vi "Update Overlay.vi"(8 "error in":errorcluster, 11 "BigMAQ in":refnum<class "BigMAQ.lvclass">) -> (0 "error out":errorcluster, 2 "Overlays":T1[](array[typedef]), 3 "BigMAQ out":refnum<class "BigMAQ.lvclass">)   [LabVIEW 2019, in "BigMAQ.lvclass"]
uses:
  BigMAQ.lvclass
  Overlay.ctl
  BigMAQ.lvclass/BigMAQ.ctl
  <vilib>/LabVIEW Open Source Project/Unicity/RandomStringGenerator/RandomStringGenerator.lvclass
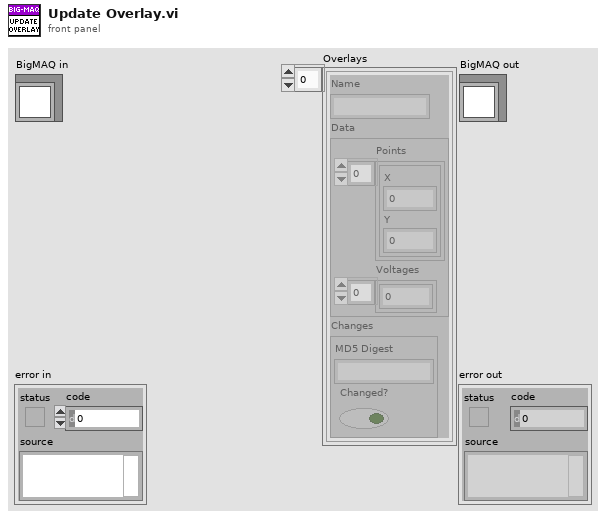
[diagram p1: front panel]
types:
  T1 = typedef "BigMAQ.lvclass/Overlay.ctl" = cluster{"Name":string, "Data":cluster{"Points":cluster{"X":dbl, "Y":dbl}[], "Voltages":dbl[]}, "Changes":cluster{"MD5 Digest":string, "Changed?":bool}}
  T2 = typedef "Image Type" = u32
  T3 = typedef "IMAQ Image.ctl" = refnum<image>
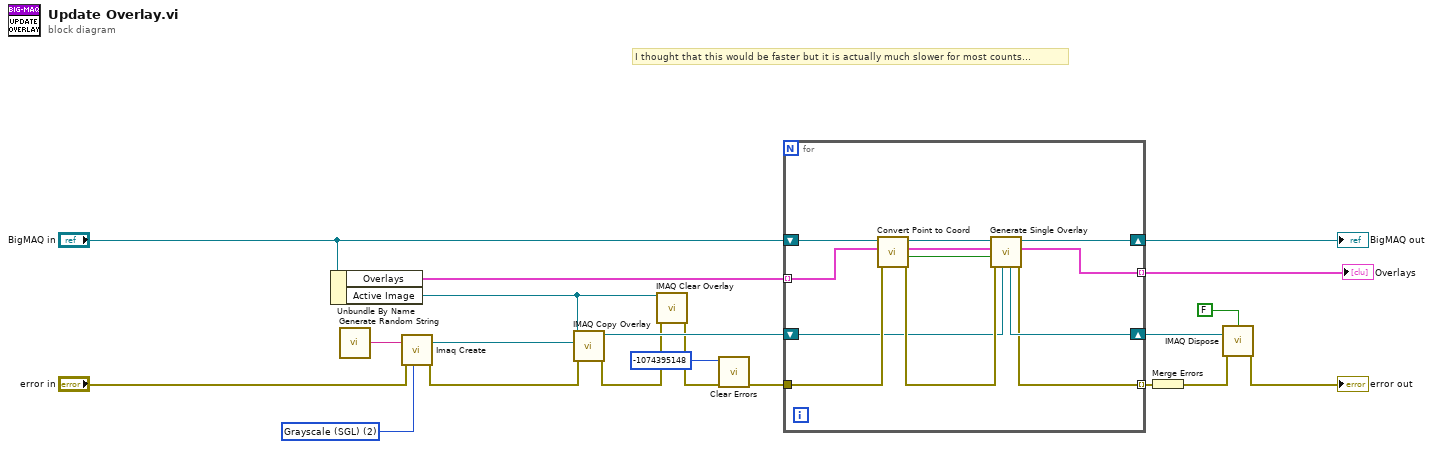
[diagram p0: block diagram]
diagram:
  w15 = T2 2 items=["Grayscale (U8)", "Grayscale (I16)", "Grayscale (SGL)", "Complex (CSG)", "RGB (U32)", "HSL (U32)", "RGB (U64)", "Grayscale (U16)"] ("Image Type")
  # "I thought that this would be faster but it is actually much slower for most counts..."
  n1 = Unbundle By Name("BigMAQ in") -> ("Overlays"=w20:T1[], "Active Image"=w5:T3)
  n2 = call <vilib>:"Generate Random String.vi"() -> ("Random String"=w13:string)  [unwired: 11 in]
  n3 = call "Imaq Create"("Image Name"=w13, "Image Type"=w15, "error in (no error)"="error in") -> ("New Image"=w12:T3, "error out"=w6:errorcluster)  [unwired: 2 in]
  n4 = call "IMAQ Copy Overlay"("error in (no error)"=w6, "Image Dst"=w12, "Image Src"=w5) -> ("error out"=w3:errorcluster, "Image Dst Out"=w11:T3)  [unwired: 7 in]
  n5 = call "IMAQ Clear Overlay"("error in (no error)"=w3, "Image"=w5) -> ("error out"=w2:errorcluster)  [unwired: 8 in, 1 out]
  n6 = call <vilib>:"Clear Errors.vi"("error in (no error)"=w2, "specific error code to clear (0: all)"=-1074395148) -> ("error out"=w4:errorcluster)  [unwired: 4 in, 1 out]
  n7 = for {
    tunnel: w20 -> [w27] mode=indexing
    tunnel: w4 -> [w25]
    tunnel: [w21] -> w19 mode=indexing
    shift-right: [w32] -> w17
    shift-left: "BigMAQ in" -> [w30]
    tunnel: [w31] -> w16 mode=indexing
    shift-right: [w22] -> w10
    shift-left: w11 -> [w23]
    n8 = call "Convert Point to Coord.vi"("error in"=w25, "Overlay"=w27, "BigMAQ in"=w30) -> ("error out"=w26:errorcluster, "Voltage Constant?"=w24:bool, "output cluster"=w28:T1, "BigMAQ out"=w29:refnum<class "BigMAQ.lvclass">)  [unwired: 5 in]
    n9 = call "Generate Single Overlay.vi"("Temp In"=w23, "error in"=w26, "Single Color"=w24, "Overlay"=w28, "BigMAQ in"=w29) -> ("error out"=w21:errorcluster, "Overlay Out"=w31:T1, "BigMAQ out"=w32:refnum<class "BigMAQ.lvclass">, "Temp Out"=w22:T3)  [unwired: 3 in]
  }
  "BigMAQ out" <- w17
  "Overlays" <- w16
  n10 = Merge Errors(w19) -> (w9:errorcluster)
  n11 = call "IMAQ Dispose"("All Images? (No)"=FALSE, "Image"=w10, "error in (no error)"=w9) -> ("error out"=→"error out":errorcluster)  [unwired: 3 in]
